vi "Register Data Handling.vi"(6 "VolatusAPI in":refnum<class "VolatusAPI.lvclass">, 8 "error in (no error)":errorcluster, 11 "LocalGraphBuffer in":refnum<class "LocalGraphBuffer.lvclass">) -> (0 "error out":errorcluster, 3 "LocalGraphBuffer out":refnum<class "LocalGraphBuffer.lvclass">)   [LabVIEW 2020, in "VolatusGUIElements.lvlib" / "LocalGraphBuffer.lvclass"]
uses:
  LocalGraphBuffer.lvclass
  C:/dev/lv20CE/relink/lv-vecto/Vecto/SubscribedDataHandler/SubscribedDataHandler.lvclass
  Volatus/VolatusAPI/VolatusAPI.lvclass
  LocalGraphBuffer.lvclass/LocalGraphBuffer.ctl
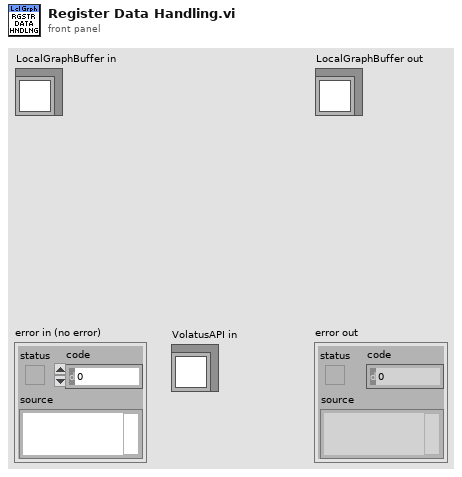
[diagram p1: front panel]
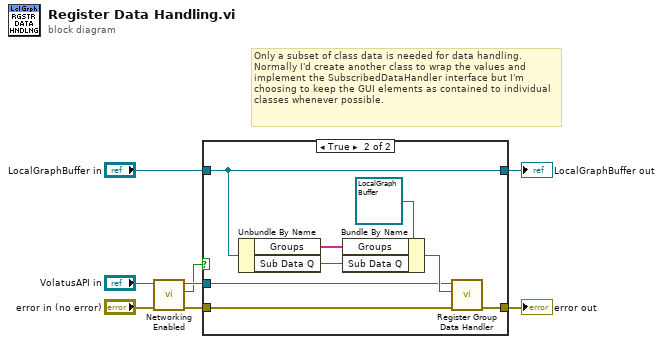
[diagram p0: block diagram]
diagram:
  # "Only a subset of class data is needed for data handling. Normally I'd create another class to wrap the values and implement the SubscribedDataHandler interface but I'm choosing to keep the GUI elements as contained to individual classes whenever possible."
  n1 = call "Networking Enabled.vi"("VolatusAPI in"="VolatusAPI in") -> ("Networking Enabled"=w1:bool, "VolatusAPI out"=w3:refnum<class "VolatusAPI.lvclass">)  [unwired: 9 in]
  n2 = case shown="True" w1 {
    tunnel: "LocalGraphBuffer in" -> [w9 w10]
    tunnel: "error in (no error)" -> [w8 w14]
    tunnel: [w8 w13] -> w5
    tunnel: w3 -> [_ w11]
    tunnel: [w9 w10] -> w2
    frame False {
    }
    frame True {
      n3 = Unbundle By Name(w10) -> ("Groups"=w12:string[], "Sub Data Q"=w16:refnum<queue>)
      n4 = Bundle By Name(cluster=refnum<class "LocalGraphBuffer.lvclass"> refnum ("LocalGraphBuffer in"), "Groups"=w12, "Sub Data Q"=w16) -> (w15:refnum<class "LocalGraphBuffer.lvclass">)
      n5 = call "Register Group Data Handler.vi"("error in (no error)"=w14, "Data Handler"=w15, "VolatusAPI in"=w11) -> ("error out"=w13:errorcluster)  [unwired: 7 in, 1 out]
    }
  }
  "error out" <- w5
  "LocalGraphBuffer out" <- w2
